vi "Evaluate Step.vi"(0 "Step Config":T4, 1 "Channel Feedback":T2, 2 "Step Phase in":T1, 3 "step start ms":dbl, 4 "dwell start ms":dbl) -> (20 "Step Phase out":T1, 21 "dwell start ms out":dbl, 22 "done":bool, 23 "passed":bool, 24 "reason":string, 25 "measured":dbl, 26 "target":dbl)   [LabVIEW 2026]
doc: "Evaluates the active step on one feedback sample; now is the feedback's timestamp_ms. Idle or Complete in: unchanged, done FALSE. Settling: timeout first (now - step start >= timeout_ms) gives Complete, done, not passed, reason Timeout; else all conditions within gives Dwell with dwell start = now. Dwell: timeout first; else not all within gives Settling; else dwell elapsed >= dwell_time_ms gives Complete, done, passed. A missing channel gives Complete, done, not passed, reason Missing channel with the channel name. measured and target come from Evaluate Conditions. Pure function, no error terminals, AF-free."
uses:
  Typedefs/Condition.ctl
  Typedefs/Channel Value.ctl
  Typedefs/Step Config.ctl
  Typedefs/Channel Feedback.ctl
  Typedefs/Step Phase.ctl
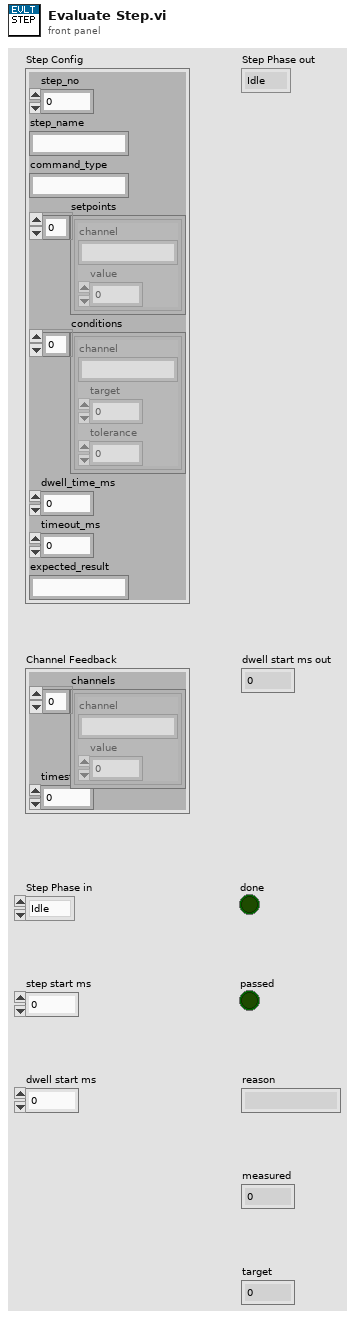
[diagram p1: front panel]
types:
  T1 = typedef "Step Phase.ctl" = enum16{"Idle", "Settling", "Dwell", "Complete"}
  T2 = typedef "Channel Feedback.ctl" = cluster{"channels":T3[], "timestamp_ms":dbl}
  T3 = typedef "Channel Value.ctl" = cluster{"channel":string, "value":dbl}
  T4 = typedef "Step Config.ctl" = cluster{"step_no":i32, "step_name":string, "command_type":string, "setpoints":T3[], "conditions":T5[], "dwell_time_ms":i32, "timeout_ms":i32, "expected_result":string}
  T5 = typedef "Condition.ctl" = cluster{"channel":string, "target":dbl, "tolerance":dbl}
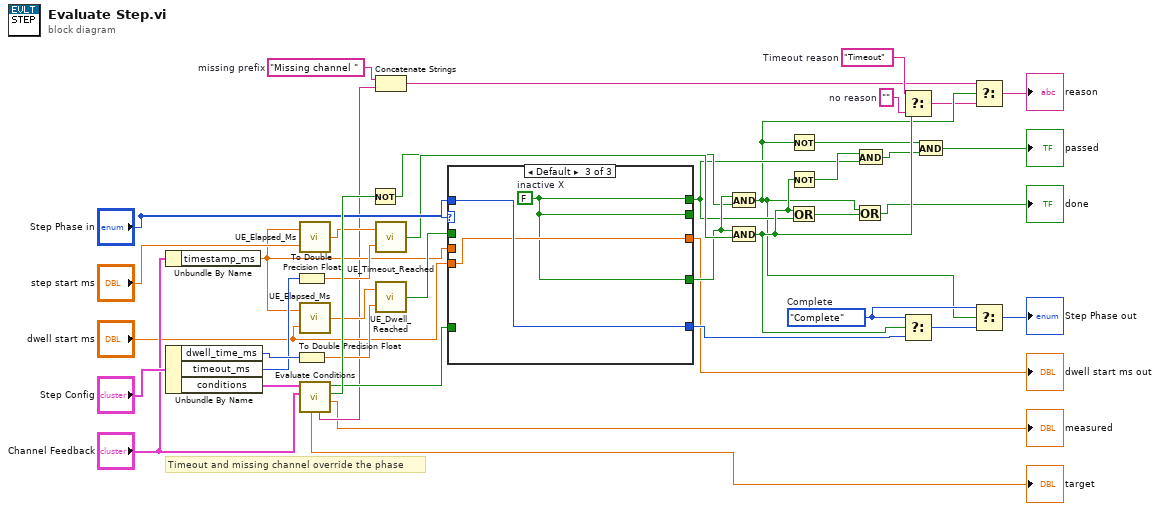
[diagram p0: block diagram]
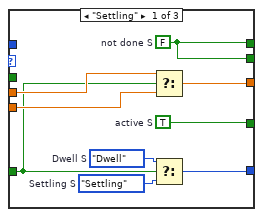
[diagram p2: hidden frame]
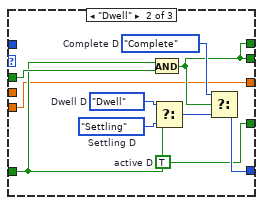
[diagram p3: hidden frame]
diagram:
  w14 = "Missing channel "  # missing prefix
  w20 = ""  # no reason
  w22 = "Timeout"  # Timeout reason
  w19 = enum16{"Idle", "Settling", "Dwell", "Complete"}."Complete"  # Complete
  # "Timeout and missing channel override the phase"
  n1 = Unbundle By Name("Channel Feedback") -> ("timestamp_ms"=w29:dbl)
  n2 = Unbundle By Name("Step Config") -> ("dwell_time_ms"=w41:i32, "timeout_ms"=w40:i32, "conditions"=w39:T5[])
  n3 = To Double Precision Float(number=w40) -> (double precision float=w34:dbl)
  n4 = To Double Precision Float(number=w41) -> (double precision float=w32:dbl)
  n5 = call "UE_Elapsed_Ms.vi"("start_ms"="step start ms", "now_ms"=w29) -> ("elapsed_ms"=w35:dbl)
  n6 = call "UE_Elapsed_Ms.vi"("start_ms"="dwell start ms", "now_ms"=w29) -> ("elapsed_ms"=w33:dbl)
  n7 = call "Evaluate Conditions.vi"("Channel Feedback"="Channel Feedback", "conditions"=w39) -> ("measured"=→"measured":dbl, "all found"=w37:bool, "all within"=w31:bool, "missing channel"=w13:string, "target"=→"target":dbl)  [unwired: 5 in]
  n8 = Not(x=w37) -> (.not. x?=w24:bool)
  n9 = Concatenate Strings(w14, w13) -> (w12:string)
  n10 = call "UE_Timeout_Reached.vi"("threshold_ms"=w34, "elapsed_ms"=w35) -> ("reached"=w26:bool)
  n11 = call "UE_Dwell_Reached.vi"("threshold_ms"=w32, "elapsed_ms"=w33) -> ("reached"=w30:bool)
  n12 = case shown="Default" "Step Phase in" {
    tunnel: "Step Phase in" -> [_ _ w64]
    tunnel: w31 -> [w48 w59 _]
    tunnel: w30 -> [_ w61 _]
    tunnel: w29 -> [w51 _ _]
    tunnel: "dwell start ms" -> [w50 w53 w63]
    tunnel: [w46 w55 w64] -> w23
    tunnel: [w45 w54 w62] -> w15
    tunnel: [w45 w54 w62] -> _
    tunnel: [w44 w53 w63] -> w6
    tunnel: [w43 w52 w62] -> w25
    frame "Settling" {
      w43 = TRUE  # active S
      w45 = FALSE  # not done S
      w47 = enum16{"Idle", "Settling", "Dwell", "Complete"}."Settling"  # Settling S
      w49 = enum16{"Idle", "Settling", "Dwell", "Complete"}."Dwell"  # Dwell S
      n13 = Select(t=w51, s=w48, f=w50) -> (s? t:f=w44:dbl)
      n14 = Select(t=w49, s=w48, f=w47) -> (s? t:f=w46:enum16{"Idle", "Settling", "Dwell", "Complete"})
    }
    frame "Dwell" {
      w52 = TRUE  # active D
      w57 = enum16{"Idle", "Settling", "Dwell", "Complete"}."Complete"  # Complete D
      w58 = enum16{"Idle", "Settling", "Dwell", "Complete"}."Settling"  # Settling D
      w60 = enum16{"Idle", "Settling", "Dwell", "Complete"}."Dwell"  # Dwell D
      n15 = And(x=w59, y=w61) -> (x .and. y?=w54:bool)
      n16 = Select(t=w60, s=w59, f=w58) -> (s? t:f=w56:enum16{"Idle", "Settling", "Dwell", "Complete"})
      n17 = Select(t=w57, s=w54, f=w56) -> (s? t:f=w55:enum16{"Idle", "Settling", "Dwell", "Complete"})
    }
    frame Default {
      w62 = FALSE  # inactive X
    }
  }
  "dwell start ms out" <- w6
  n18 = And(x=w25, y=w24) -> (x .and. y?=w11:bool)
  n19 = And(x=w25, y=w26) -> (x .and. y?=w21:bool)
  n20 = Not(x=w11) -> (.not. x?=w9:bool)
  n21 = Not(x=w21) -> (.not. x?=w16:bool)
  n22 = Or(x=w21, y=w15) -> (x .or. y?=w17:bool)
  n23 = Or(x=w11, y=w17) -> (x .or. y?=→"done":bool)
  n24 = And(x=w16, y=w15) -> (x .and. y?=w8:bool)
  n25 = Select(t=w22, s=w21, f=w20) -> (s? t:f=w10:string)
  n26 = Select(t=w19, s=w21, f=w23) -> (s? t:f=w18:T1)
  n27 = And(x=w9, y=w8) -> (x .and. y?=→"passed":bool)
  n28 = Select(t=w12, s=w11, f=w10) -> (s? t:f=→"reason":string)
  n29 = Select(t=w19, s=w11, f=w18) -> (s? t:f=→"Step Phase out":T1)
